vi "Example - Hello World.vi"() -> ()   [LabVIEW 2019]
uses:
  src/KoRE-MQTT.lvlib
  src/KoRE-MQTT/Public/TypeDefs/MQTT Version.ctl
panel:
  in  "Version":T1=4 items=["3.11"=4, "5.0"=5]
  out "Sent?":bool
  in  "Port":u16=1883
  in  "Password":string
  in  "Username":string
  out "Received topic":string
  out "Received?":bool
  out "Send to topic":string
  out "Received message":string
  in  "Message":string="Hello properties!"
  in  "Host":string(combo)="test.mosquitto.org"
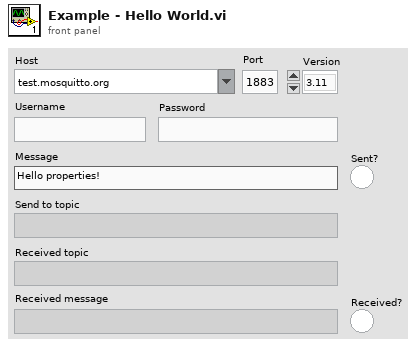
[diagram p1: front panel]
types:
  T1 = typedef "KoRE-MQTT.lvlib/MQTT Version.ctl" = u16
  T2 = typedef "KoRE-MQTT.lvlib/MQTT Refnum.ctl" = refnum<vi>
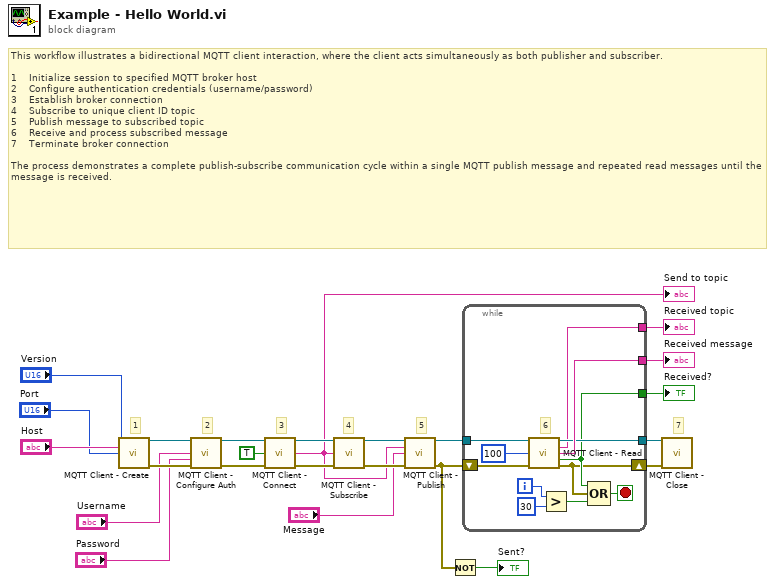
[diagram p0: block diagram]
diagram:
  # "7"
  # "5"
  # "This workflow illustrates a bidirectional MQTT client interaction, where the client acts simultaneously as both publisher and subscriber.\n\n1    Initialize session to specified MQTT broker host\n2    Configure authentication credentials (username/password)\n3    Establish broker connection\n4    Subscribe to unique client ID topic\n5    Publish message to subscribed topic\n6    Receive and process subscribed message\n7    Terminate broker connection\n\nThe process demonstrates a complete publish-subscribe communication cycle within a single MQTT publish message and repeated read messages until the message is received."
  # "4"
  # "3"
  # "2"
  # "1"
  n1 = call "MQTT Client - Create.vi"("Version (3.11)"="Version", "Host"="Host", "Port (1883)"="Port") -> ("MQTT Session"=w9:T2, "error out"=w10:errorcluster)  [unwired: 11 in]
  n2 = call "MQTT Client - Configure Auth.vi"("MQTT Session"=w9, "Username"="Username", "Password"="Password", "error in (no error)"=w10) -> ("MQTT Session out"=w8:T2, "error out"=w7:errorcluster)  [unwired: 10 in]
  n3 = call "MQTT Client - Connect.vi"("MQTT Session"=w8, "Clean Start"=TRUE, "error in (no error)"=w7) -> ("MQTT Session out"=w24:T2, "Assigned Client Identifier"=w12:string, "error out"=w23:errorcluster)  [unwired: 8 in, 2 out]
  "Send to topic" <- w12
  n4 = call "MQTT Client - Subscribe.vi"("MQTT Session"=w24, "Single Topic Filter"=w12, "error in (no error)"=w23) -> ("MQTT Session out"=w20:T2, "error out"=w21:errorcluster)  [unwired: 11 in]
  n5 = call "MQTT Client - Publish.vi"("MQTT Session"=w20, "Topic"=w12, "Message"="Message", "error in"=w21) -> ("MQTT Session out"=w18:T2, "error out"=w2:errorcluster)  [unwired: 10 in]
  n6 = Not(x=w2) -> (.not. x?=→"Sent?":bool)
  n7 = while {
    shift-right: [w26] -> w19
    shift-left: w2 -> [w30]
    tunnel: w18 -> [w35]
    tunnel: [w32] -> w17
    tunnel: [w31] -> w16
    tunnel: [w27] -> w15
    tunnel: [w29] -> w11
    i -> [w34]
    stop <- w25 stop-if-true
    # "6"
    n8 = call "MQTT Client - Read.vi"("MQTT Session"=w35, "timeout (global)"=100, "error in (no error)"=w30) -> ("MQTT Session out"=w31:T2, "Topic"=w29:string, "Message"=w32:string, "New message?"=w27:bool, "error out"=w26:errorcluster)  [unwired: 6 in, 2 out]
    n9 = Greater?(x=w34, y=30) -> (0:w28:bool)
    n10 = Compound Arithmetic op=OR(w27, w26, w28) -> (w25:bool)
  }
  "Received message" <- w17
  "Received?" <- w15
  "Received topic" <- w11
  n11 = call "MQTT Client - Close.vi"("MQTT session"=w16, "error in (no error)"=w19) -> ()  [unwired: 13 in, 1 out]
